vi "Controls - By List.vi"(7 "Msg Chain":string, 8 "error in (no error)":errorcluster {"code" format="Error %.0f"}, 10 "Controls Docs":refnum<class "GUI Documentation.lvclass">[](array[class]), 11 "VIDoc Printer - Confluence In":refnum<class "VIDoc Printer - Confluence.lvclass">) -> (0 "error out":errorcluster {"code" format="Error %.0f"}, 3 "VIDoc Printer - Confluence Out":refnum<class "VIDoc Printer - Confluence.lvclass">)   [LabVIEW 2023, in "VIDoc Printer - Confluence.lvlib" / "VIDoc Printer - Confluence.lvclass"]
uses:
  VIDoc Printer - Confluence.lvclass
  <vilib>/DMC/VIDoc/Framework/Parsing/GUI Documentation/GUI Documentation.lvclass
  Confluence Formatting/Types/Format Combo Box.ctl
  <vilib>/DMC/VIDoc/Framework/Printer/VIDoc Printer.lvclass/VIDoc Printer.ctl
  VIDoc Printer - Confluence.lvclass/VIDoc Printer - Confluence.ctl
  <vilib>/DMC/VIDoc/Framework/Parsing/GUI Documentation/GUI Documentation.lvclass/GUI Documentation.ctl
  Types/VI Method Types.ctl
  <vilib>/DMC/VIDoc/Framework/Parsing/GUI Documentation/Get VI Info.vi
  <vilib>/DMC/VIDoc/Framework/Printer/Accessors/Get Formatting Settings - Bookmark Options.vi
  <vilib>/DMC/VIDoc/Framework/Printer/Accessors/Get Controls Settings - List Detail Level.vi
  Accessors/Get Sortable Tables.vi
  Accessors/Get Temporary Image Directory+.vi
  Accessors/Get Ctrls By List Expand.vi
  <vilib>/Utility/libraryn.llb/Create Directory Recursive.vi
  Confluence Formatting/Confluence Formatting.lvlib
  <vilib>/DMC/VIDoc/Framework/Printer/VIDoc Printer.lvclass
  <vilib>/DMC/VIDoc/Framework/UI Interaction/Interface/UI Interaction.lvclass
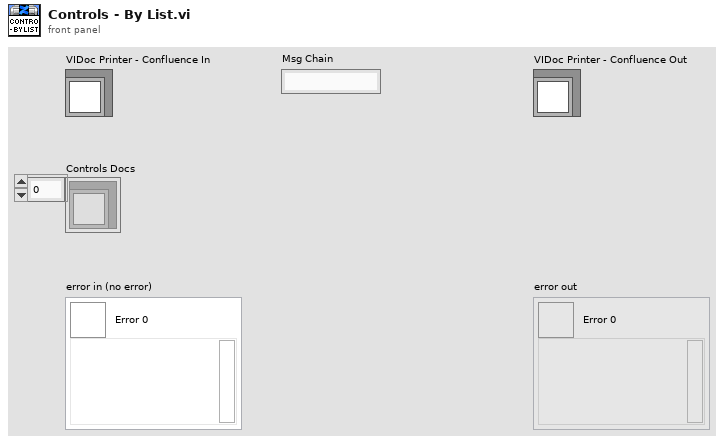
[diagram p1: front panel]
types:
  T1 = typedef "Confluence Formatting.lvlib/Format Combo Box.ctl" = string
  T2 = typedef "VIDoc Printer.lvlib/Printer Settings.lvclass/Bookmark Options.ctl" = cluster{"Bookmarks as New Line in VI Descriptions":bool, "Unique Bookmark Tags Only":bool, "Include Tag and Text":bool}
  T3 = typedef "VIDoc Printer.lvlib/Printer Settings.lvclass/Detail Level Enum.ctl" = enum16{"None", "Minimal", "Standard", "Full"}
  T4 = typedef "VIDoc Printer - Confluence.lvlib/VIDoc Printer - Confluence.lvclass/VI Method Types.ctl" = enum16{"Library", "Class", "Interface", "LLB", "UI", "List"}
  T5 = typedef "VIDoc Parsing.lvlib/Method Spec Cluster.ctl" = cluster{"VI Type Ext":T6, "Name":string, "Path":path, "Get Conpane Image":T7, "Description":string, "Get Library Access Scope":enum32{"invalid scope", "public", "private", "protected", "community"}, "Dispatch":T8, "ContainsCompiledCode":bool, "Exec.IsReentrant":bool, "Exec.ReentrancyType":enum16{"Share clones between instances", "Preallocate clone for each instance"}, "ExecInlining":bool, "ExecInlineIfPossible":bool, "Auto Err Handling":bool, "CodeComplexity":sgl, "Bookmark Tags":string[], "Control VI Type":enum32{"not a control VI", "control", "typedef", "strict typedef"}, "Controls":T9[], "VI Type":enum32{"invalid VI type", "Standard VI", "Control VI", "Global VI", "Polymorphic VI", "Configuration VI", "SubSystem", "Facade VI", "Method VI", "Statechart Diagram VI"}, "Minimum Size":T11, "Front Panel Window:Title":string, "Front Panel Window:Behavior":enum32{"Invalid", "Default", "Floating", "Floating/Auto-Hide", "Modal"}, "Front Panel Window:Closeable":bool, "Must Override":bool, "Must Use Parent Implementation":bool, "VI Icon":T7, "Front Panel":T7, "History:Revision Number":u32, "Metrics:Total Data Size":u32, "Execution:Allow Debugging":bool, "Execution:Preferred Exec System":enum32{"invalid execution system", "user interface", "standard", "instrument i/o", "data acquisition", "other 1", "other 2", "same as caller"}, "Execution:Priority":enum32{"invalid priority", "background priority", "normal priority", "above normal priority", "high priority", "time critical priority", "subroutine"}, "BM Tag Text":string[], "Block Diagram":T7, "Structure Tree":T12[]}
  T6 = typedef "VIDoc Parsing.lvlib/VI Type Extended Enum.ctl" = enum16{"Unknown", "Class Method", "Class Accessor Get", "Class Accessor Set", "Class Control", "Library Method", "Library Control", "VI", "Control"}
  T7 = typedef "imagedata.ctl" = cluster{"image type":i32, "image depth":i32, "image":u8[], "mask":u8[], "colors":u32[], "Rectangle":cluster{"left":i16, "top":i16, "right":i16, "bottom":i16}}
  T8 = typedef "VIDoc Parsing.lvlib/Class Dispatch Type Enum.ctl" = enum16{"None", "Static", "Dynamic"}
  T9 = typedef "VIDoc Parsing.lvlib/Controls Info Cluster.ctl" = cluster{"Name":string, "Description":string, "Data Type":string, "Tip Strip":string, "UID":i32, "Image Data":T7, "ToggleKeyBind":T10, "Raw Label":string, "Raw Caption":string}
  T10 = typedef "LVKeyTypeDef.ctl" = cluster{"Focus":bool, "Control":bool, "Shift":bool, "Key":string}
  T11 = typedef "LVPointTypeDef.ctl" = cluster{"Horizontal":i16, "Vertical":i16}
  T12 = typedef "VIDoc Parsing.lvlib/Structure Reporter.lvlib/Tree Cluster.ctl" = cluster{"Object Class Name":string, "Labels":string[], "Child Tag":string, "Item Indent":i32, "Child Only?":bool, "Glyph Index":i32}
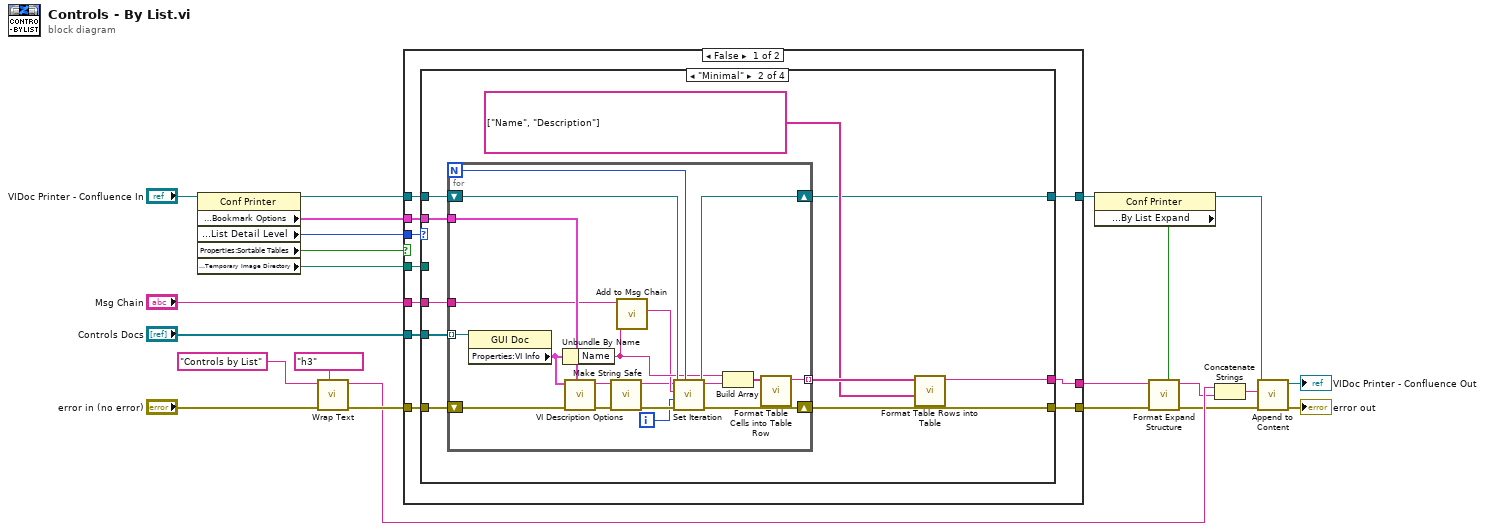
[diagram p0: block diagram]
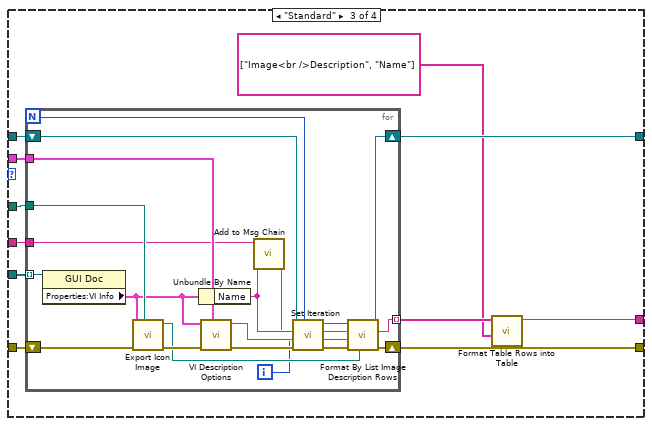
[diagram p3: hidden frame]
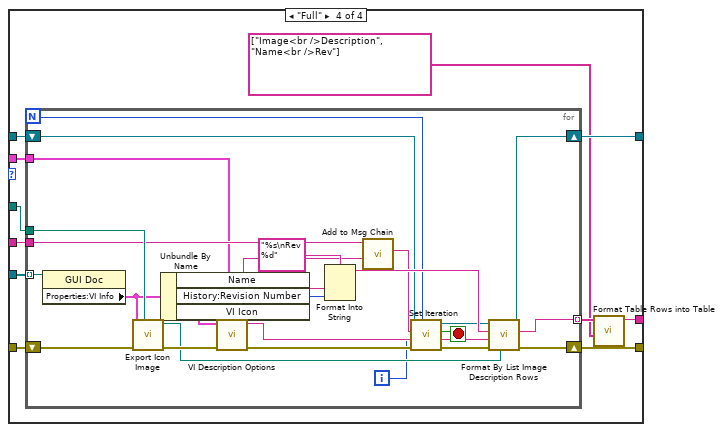
[diagram p4: hidden frame]
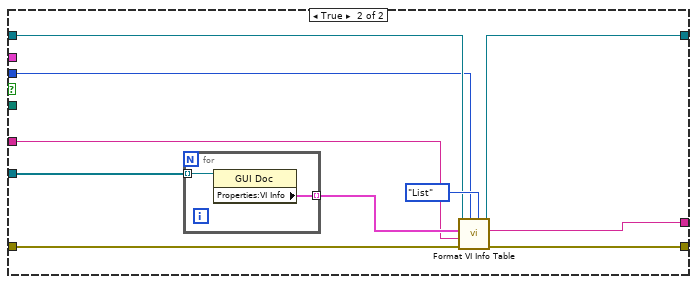
[diagram p5: hidden frame]
diagram:
  n1 = property class="Conf Printer"(reference="VIDoc Printer - Confluence In") -> (reference out=w20:refnum<class "VIDoc Printer - Confluence.lvclass">, "Properties:Settings:Formatting Options:Bookmark Options"=w9:T2, "Properties:Settings:Control Members:List Detail Level"=w8:T3, "Properties:Sortable Tables"=w2:bool, "Properties:Temporary Image Directory"=w1:path)  [unwired: 1 in, 1 out]
  n2 = call "Wrap Text.vi"("Formatting"=T1 "h3", "Error in"="error in (no error)", "String"="Controls by List" ("format string")) -> ("Error out"=w22:errorcluster, "Wrapped String"=w17:string)  [unwired: 7 in]
  n3 = case shown="False" w2 {
    tunnel: w22 -> [w33 w136]
    tunnel: [w32 w135] -> w21
    tunnel: w20 -> [w31 w133]
    tunnel: [w30 w129] -> w19
    tunnel: w1 -> [w29 _]
    tunnel: "Controls Docs" -> [w28 w130]
    tunnel: "Msg Chain" -> [w27 w131]
    tunnel: w9 -> [w26 _]
    tunnel: w8 -> [w25 w132]
    tunnel: [w24 w134] -> w6
    frame False {
      n4 = case shown="\"Minimal\"" w25 {
        tunnel: w33 -> [w35 w44 w72 w103]
        tunnel: [w35 w41 w66 w97] -> w32
        tunnel: w28 -> [_ w45 w73 w104]
        tunnel: [_ w42 w68 w99] -> w24
        tunnel: w31 -> [w34 w39 w70 w101]
        tunnel: [w34 w38 w69 w100] -> w30
        tunnel: w29 -> [_ _ w71 w102]
        tunnel: w27 -> [_ w37 w64 w95]
        tunnel: w26 -> [_ w36 w63 w94]
        frame "None", Default {
        }
        frame "Minimal" {
          n5 = for {
            N -> [w51]
            tunnel: w45 -> [w62] mode=indexing
            tunnel: w36 -> [w60]
            shift-right: [w54] -> w41
            shift-left: w44 -> [w59]
            tunnel: [w56] -> w43 mode=indexing
            shift-right: [w52] -> w38
            shift-left: w39 -> [w53]
            tunnel: w37 -> [w49]
            i -> [w50]
            n6 = property class="GUI Doc"(reference=w62) -> ("Properties:VI Info"=w61:T5)  [unwired: 1 in, 2 out]
            n7 = Unbundle By Name(w61) -> ("Name"=w48:string)
            n8 = call <vilib>:"VI Description Options.vi"("Bookmark Options"=w60, "Error in"=w59, "VI Info"=w61) -> ("Error out"=w55:errorcluster, "Description"=w58:string)  [unwired: 7 in]
            n9 = call "Make String Safe.vi"("Raw String"=w58) -> ("String out"=w46:string)  [unwired: 9 in, 1 out]
            n10 = call <vilib>:"Add to Msg Chain.vi"("New"=w48, "Msg Chain in"=w49) -> ("Msg Chain out"=w47:string)  [unwired: 9 in]
            n11 = call <vilib>:"Set Iteration.vi"("Progress Max"=w51, "error in (no error)"=w55, "Progress Value"=w50, "Message (No Message Update)"=w47, "VIDoc Printer In"=w53) -> ("error out"=w54:errorcluster, "VIDoc Printer Out"=w52:refnum<class "VIDoc Printer - Confluence.lvclass">)  [unwired: 4 in, 1 out]
            n12 = Build Array(w48, w46) -> (w57:string[])
            n13 = call "Format Table Cells into Table Row.vi"("Table Cells"=w57) -> ("Table Row Text"=w56:string)  [unwired: 10 in]
          }
          n14 = call "Format Table Rows into Table.vi"("Table Headers"=string[] ["Name", "Description"], "Table Rows"=w43) -> ("Table Text"=w42:string)  [unwired: 9 in]
        }
        frame "Standard" {
          n15 = for {
            N -> [w78]
            tunnel: w73 -> [w93] mode=indexing
            tunnel: w63 -> [w92]
            shift-right: [w87] -> w66
            shift-left: w72 -> [w90]
            tunnel: w71 -> [w91]
            shift-right: [w86] -> w69
            shift-left: w70 -> [w80]
            tunnel: [w83] -> w67 mode=indexing
            tunnel: w64 -> [w76]
            i -> [w77]
            n16 = property class="GUI Doc"(reference=w93) -> ("Properties:VI Info"=w88:T5)  [unwired: 1 in, 2 out]
            n17 = call <vilib>:"Export Icon Image.vi"("Temporary Image Directory"=w91, "Error in"=w90, "VI Info"=w88) -> ("Error out"=w89:errorcluster, "Image Path"=w84:path)  [unwired: 7 in]
            n18 = Unbundle By Name(w88) -> ("Name"=w75:string)
            n19 = call <vilib>:"VI Description Options.vi"("Bookmark Options"=w92, "Error in"=w89, "VI Info"=w88) -> ("Error out"=w82:errorcluster, "Description"=w85:string)  [unwired: 7 in]
            n20 = call <vilib>:"Add to Msg Chain.vi"("New"=w75, "Msg Chain in"=w76) -> ("Msg Chain out"=w74:string)  [unwired: 9 in]
            n21 = call <vilib>:"Set Iteration.vi"("Progress Max"=w78, "error in (no error)"=w82, "Progress Value"=w77, "Message (No Message Update)"=w74, "VIDoc Printer In"=w80) -> ("error out"=w81:errorcluster, "VIDoc Printer Out"=w79:refnum<class "VIDoc Printer - Confluence.lvclass">)  [unwired: 4 in, 1 out]
            n22 = call "Format By List Image Description Rows.vi"("Image"=w84, "error in (no error)"=w81, "Description"=w85, "Name"=w75, "VIDoc Printer - Confluence In"=w79) -> ("error out"=w87:errorcluster, "Table Rows Text"=w83:string, "VIDoc Printer - Confluence Out"=w86:refnum<class "VIDoc Printer - Confluence.lvclass">)  [unwired: 3 in, 1 out]
          }
          n23 = call "Format Table Rows into Table.vi"("Table Headers"=string[] ["Image<br />Description", "Name"], "Table Rows"=w67) -> ("Table Text"=w68:string)  [unwired: 9 in]
        }
        frame "Full" {
          n24 = for {
            N -> [w111]
            tunnel: w104 -> [w128] mode=indexing
            shift-right: [w123] -> w97
            shift-left: w103 -> [w126]
            tunnel: w102 -> [w127]
            shift-right: [w122] -> w100
            shift-left: w101 -> [w113]
            tunnel: [w119] -> w98 mode=indexing
            tunnel: w95 -> [w109]
            tunnel: w94 -> [w105]
            i -> [w110]
            stop <- w106 stop-if-true
            n25 = property class="GUI Doc"(reference=w128) -> ("Properties:VI Info"=w124:T5)  [unwired: 1 in, 2 out]
            n26 = call <vilib>:"Export Icon Image.vi"("Temporary Image Directory"=w127, "Error in"=w126, "VI Info"=w124) -> ("Error out"=w125:errorcluster, "Image Path"=w120:path)  [unwired: 7 in]
            n27 = Unbundle By Name(w124) -> ("Name"=w108:string, "History:Revision Number"=w117:u32)  [unwired: 1 out]
            n28 = call <vilib>:"VI Description Options.vi"("Bookmark Options"=w105, "Error in"=w125, "VI Info"=w124) -> ("Error out"=w115:errorcluster, "Description"=w121:string)  [unwired: 7 in]
            n29 = Format Into String(format string="%s\nRev %d", w108, w117) -> (resulting string=w116:string)  [unwired: 2 in, 1 out]
            n30 = call <vilib>:"Add to Msg Chain.vi"("New"=w108, "Msg Chain in"=w109) -> ("Msg Chain out"=w107:string)  [unwired: 9 in]
            n31 = call <vilib>:"Set Iteration.vi"("Progress Max"=w111, "error in (no error)"=w115, "Progress Value"=w110, "Message (No Message Update)"=w107, "VIDoc Printer In"=w113) -> ("error out"=w114:errorcluster, "Abort?"=w106:bool, "VIDoc Printer Out"=w112:refnum<class "VIDoc Printer - Confluence.lvclass">)  [unwired: 4 in]
            n32 = call "Format By List Image Description Rows.vi"("Image"=w120, "error in (no error)"=w114, "Description"=w121, "Name"=w116, "VIDoc Printer - Confluence In"=w112) -> ("error out"=w123:errorcluster, "Table Rows Text"=w119:string, "VIDoc Printer - Confluence Out"=w122:refnum<class "VIDoc Printer - Confluence.lvclass">)  [unwired: 3 in, 1 out]
          }
          n33 = call "Format Table Rows into Table.vi"("Table Headers"=string[] ["Image<br />Description", "Name<br />Rev"], "Table Rows"=w98) -> ("Table Text"=w99:string)  [unwired: 9 in]
        }
      }
    }
    frame True {
      n34 = for {
        tunnel: w130 -> [w140] mode=indexing
        tunnel: [w139] -> w137 mode=indexing
        n35 = property class="GUI Doc"(reference=w140) -> ("Properties:VI Info"=w139:T5)  [unwired: 1 in, 2 out]
      }
      n36 = call "Format VI Info Table.vi"("Type"=VI_Method_Types."List", "Methods"=w132, "Error in"=w136, "Msg Chain"=w131, "VI Info Array"=w137, "VIDoc Printer - Confluence In"=w133) -> ("Error out"=w135:errorcluster, "Table String"=w134:string, "VIDoc Printer - Confluence Out"=w129:refnum<class "VIDoc Printer - Confluence.lvclass">)  [unwired: 3 in]
    }
  }
  n37 = property class="Conf Printer"(reference=w19) -> (reference out=w4:refnum<class "VIDoc Printer - Confluence.lvclass">, "Properties:Expand?:Control:By List Expand"=w3:bool)  [unwired: 1 in, 1 out]
  n38 = call "Format Expand Structure.vi"("Enable? (T)"=w3, "Error in"=w21, "Content"=w6) -> ("Error out"=w7:errorcluster, "Expand String"=w5:string)  [unwired: 7 in]
  n39 = Concatenate Strings(w17, w5) -> (w18:string)
  n40 = call "Append to Content.vi"("error in (no error)"=w7, "Content"=w18, "VIDoc Printer - Confluence In"=w4) -> ("error out"=→"error out":errorcluster, "VIDoc Printer - Confluence Out"=→"VIDoc Printer - Confluence Out":refnum<class "VIDoc Printer - Confluence.lvclass">)  [unwired: 7 in]
